vi "close.vi"(8 "error in":errorcluster, 11 "Shared Memory runtime in":refnum<class "Shared Memory runtime.lvclass">) -> (0 "error out":errorcluster)   [LabVIEW 2014, in "Shared Memory runtime.lvclass"]
doc: "Provides an interface for terminating a module instance. While this interface performs no operations, a child should close and deallocate any open references or memory."
uses:
  Shared Memory runtime.lvclass
  Shared Memory runtime.lvclass/Shared Memory runtime.ctl
  <vilib>/NI/NI Linux RT IPC/Shared Memory/Classes/Shared Memory/Shared Memory.lvclass
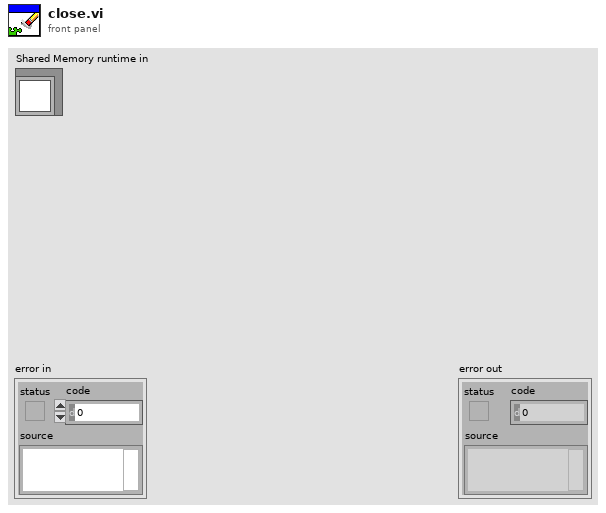
[diagram p1: front panel]
types:
  T1 = typedef "Shared Memory runtime.lvclass/channel runtime.ctl" = cluster{"channel classification":T2, "data type":T3, "pointer to shared memory":u64, "number of elements":u64, "data dictionary index":cluster{i32[]}, "shared memory":T4, "first tag index":i32, "sequential tags?":bool}
  T2 = typedef "TBM channel.lvclass/channel classification.ctl" = enum16{"input data", "output data", "processing parameter", "processing result"}
  T3 = typedef "tag bus.lvlib/tag descriptor.lvclass/Data Type.ctl" = enum16{"Double", "Single", "I64", "I32", "I16", "I8", "U64", "U32", "U16", "U8", "Boolean", "String", "Array of Double", "Array of Single", "Array of I64", "Array of I32", "Array of I16", "Array of I8", "Array of U64", "Array of U32", "Array of U16", "Array of U8", "Array of Boolean", "Array of String"}
  T4 = typedef "Linux RT IPC.Shared Memory.lvlib/reference.ctl" = refnum<data-value>
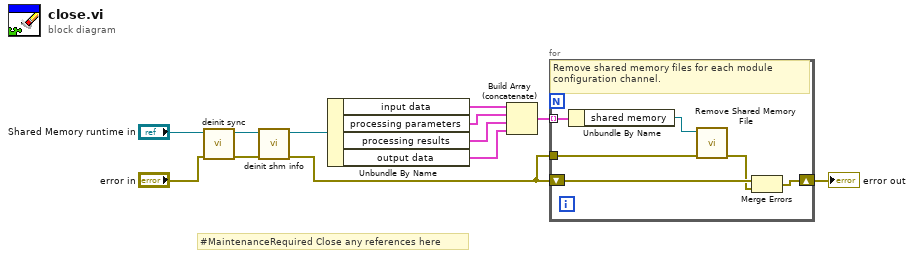
[diagram p0: block diagram]
diagram:
  # "#MaintenanceRequired Close any references here"
  n1 = call "deinit sync.vi"("error in (no error)"="error in", "Shared Memory runtime in"="Shared Memory runtime in") -> ("error out"=w3:errorcluster, "Shared Memory runtime out"=w4:refnum<class "Shared Memory runtime.lvclass">)  [unwired: 8 in]
  n2 = call "deinit shm info.vi"("error in (no error)"=w3, "Shared Memory runtime in"=w4) -> ("error out"=w2:errorcluster, "Shared Memory runtime out"=w1:refnum<class "Shared Memory runtime.lvclass">)  [unwired: 8 in]
  n3 = Unbundle By Name(w1) -> ("input data"=w12:T1[], "processing parameters"=w11:T1[], "processing results"=w10:T1[], "output data"=w9:T1[])
  n4 = Build Array (concatenate)(w12, w11, w10, w9) -> (w8:T1[])
  n5 = for {
    tunnel: w8 -> [w18] mode=indexing
    shift-right: [w13] -> w7
    shift-left: w2 -> [w15]
    tunnel: w2 -> [w16]
    # "Remove shared memory files for each module configuration channel."
    n6 = Unbundle By Name(w18) -> ("shared memory"=w17:T4)
    n7 = call <vilib>:"Remove Shared Memory File.vi"("error in (no error)"=w16, "shared memory in"=w17) -> ("error out"=w14:errorcluster)  [unwired: 8 in, 1 out]
    n8 = Merge Errors(w15, w14) -> (w13:errorcluster)
  }
  "error out" <- w7
